vi "Elevator Test Bench.vi"() -> ()   [LabVIEW 2021]
uses:
  Elevator/Elevator.lvclass
  DAQNavi_AI.lvclass/DAQNavi_AI.lvclass
  C:/Users/lincoln.lucio/Documents/Lincoln/Documentos Pessoais/meus docs/Projetos pessoais/Projeto Sciranda/projeto_versioned/sciranda/AnalogInput/AnalogInput.lvclass
  DAQNavi_AO.lvclass/DAQNavi_AO.lvclass
  C:/Users/lincoln.lucio/Documents/Lincoln/Documentos Pessoais/meus docs/Projetos pessoais/Projeto Sciranda/projeto_versioned/sciranda/AnalogOutput/AnalogOutput.lvclass
  DAQNavi_AO.lvclass/DAQNavi_AO.lvclass/DAQNavi_AO.ctl
  DAQNavi_AI.lvclass/DAQNavi_AI.lvclass/DAQNavi_AI.ctl
panel:
  out "Actual Position":dbl
  in  "Elevator Position Control":dbl
  in  "stop":bool
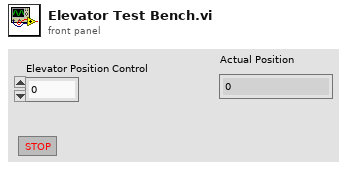
[diagram p1: front panel]
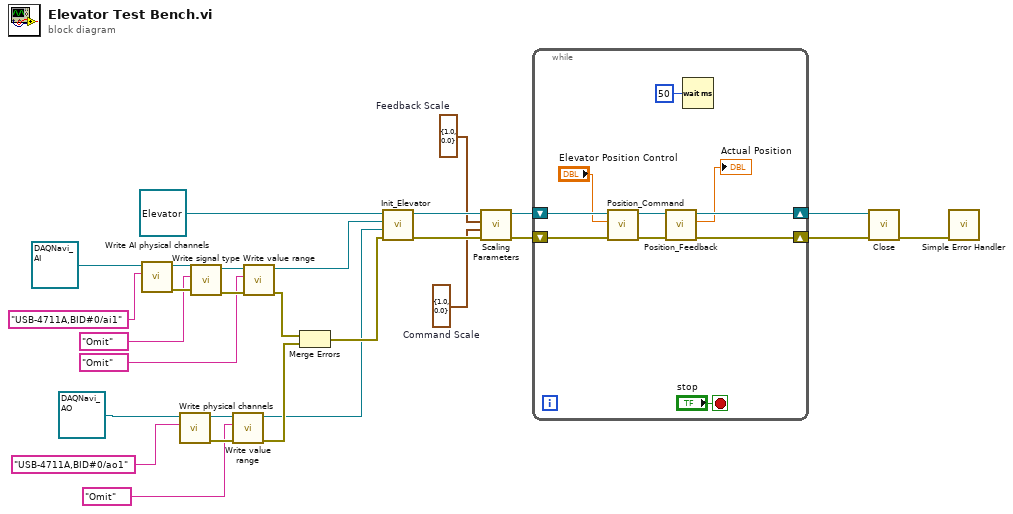
[diagram p0: block diagram]
diagram:
  w20 = cluster{"Output_Gain":dbl, "Output_Offset":dbl} {"Output_Gain"=1.0, "Output_Offset"=0.0}  # Command Scale
  w21 = cluster{"Input_Gain":dbl, "Input_Offset":dbl} {"Input_Gain"=1.0, "Input_Offset"=0.0}  # Feedback Scale
  n1 = call "Write AI physical channels.vi"("physical channels"="USB-4711A,BID#0/ai1", "DAQNavi_AI in"=refnum<class "DAQNavi_AI.lvclass"> refnum ("DAQNavi_AI.lvclass")) -> ("error out"=w17:errorcluster, "DAQNavi_AI out"=w18:refnum<class "DAQNavi_AI.lvclass">)  [unwired: 8 in]
  n2 = call "Write physical channels.vi"("physical channels"="USB-4711A,BID#0/ao1", "DAQNavi_AO in"=refnum<class "DAQNavi_AO.lvclass"> refnum ("DAQNavi_AO.lvclass")) -> ("error out"=w9:errorcluster, "DAQNavi_AO out"=w10:refnum<class "DAQNavi_AO.lvclass">)  [unwired: 8 in]
  n3 = call "Write signal type.vi"("error in (no error)"=w17, "signal type"="Omit", "DAQNavi_AI in"=w18) -> ("error out"=w15:errorcluster, "DAQNavi_AI out"=w16:refnum<class "DAQNavi_AI.lvclass">)  [unwired: 7 in]
  n4 = call "Write value range.vi"("error in (no error)"=w9, "value range"="Omit", "DAQNavi_AO in"=w10) -> ("error out"=w4:errorcluster, "DAQNavi_AO out"=w1:refnum<class "DAQNavi_AO.lvclass">)  [unwired: 7 in]
  n5 = call "Write value range.vi"("error in (no error)"=w15, "value range"="Omit", "DAQNavi_AI in"=w16) -> ("error out"=w5:errorcluster, "DAQNavi_AI out"=w2:refnum<class "DAQNavi_AI.lvclass">)  [unwired: 7 in]
  n6 = Merge Errors(w5, w4) -> (w3:errorcluster)
  n7 = call "Init_Elevator.vi"("error in (no error)"=w3, "AnalogOutput.lvclass"=w1, "AnalogInput.lvclass"=w2, "Elevator in"=refnum<class "Elevator.lvclass"> refnum) -> ("error out"=w27:errorcluster, "Elevator out"=w28:refnum<class "Elevator.lvclass">)  [unwired: 6 in]
  n8 = call "Scaling Parameters.vi"("error in (no error)"=w27, "Command Scale"=w20, "Feedback Scale"=w21, "Elevator in"=w28) -> ("error out"=w25:errorcluster, "Elevator out"=w26:refnum<class "Elevator.lvclass">)  [unwired: 6 in]
  n9 = while {
    shift-right: [w34] -> w24
    shift-left: w26 -> [w38]
    shift-right: [w33] -> w23
    shift-left: w25 -> [w37]
    stop <- "stop" stop-if-true
    n10 = call "Position_Command.vi"("error in (no error)"=w37, "Elevator Position Control"="Elevator Position Control", "Elevator in"=w38) -> ("error out"=w35:errorcluster, "Elevator out"=w36:refnum<class "Elevator.lvclass">)  [unwired: 7 in]
    n11 = call-dynamic "Position_Feedback.vi"("error in (no error)"=w35, "Elevator in"=w36) -> ("error out"=w33:errorcluster, "Actual Position"=→"Actual Position":dbl, "Elevator out"=w34:refnum<class "Elevator.lvclass">)  [unwired: 7 in]
    n12 = Wait (ms)(milliseconds to wait=u32 50) -> ()  [unwired: 1 out]
  }
  n13 = call-dynamic "Close.vi"("error in (no error)"=w23, "Elevator in"=w24) -> ("error out"=w19:errorcluster)  [unwired: 8 in, 1 out]
  n14 = call <vilib>:"Simple Error Handler.vi"("error in (no error)"=w19) -> ()  [unwired: 4 in, 5 out]
